vi "Get User Reference by Name.vi"(4 "error in (no error)":errorcluster, 6 "LoginName":string, 7 "EasyUserManager in":refnum<class "EasyUserManager.lvclass">) -> (0 "error out":errorcluster, 2 "User Reference":refnum<k7>, 3 "EasyUserManager out":refnum<class "EasyUserManager.lvclass">)   [LabVIEW 2024, in "EasyUserManager.lvclass"]
doc: "Returns the <B>User Reference</B> corresponding to the provided <B>LoginName</B>. \n\nYou must close the reference after using it."
uses:
  EasyUserManager.lvclass
  EasyUserManager.lvclass/EasyUserManager.ctl
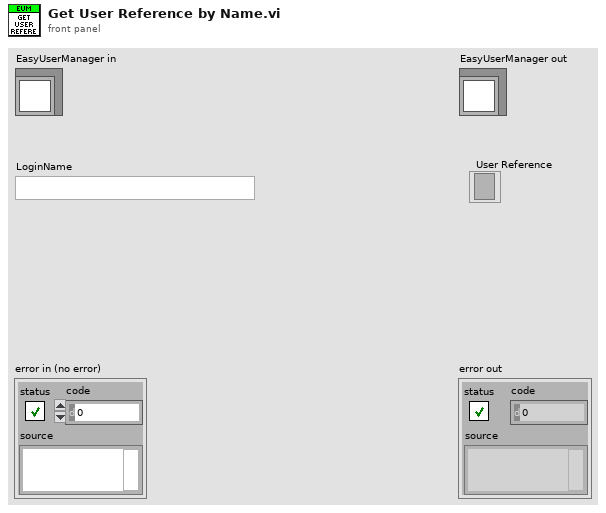
[diagram p1: front panel]
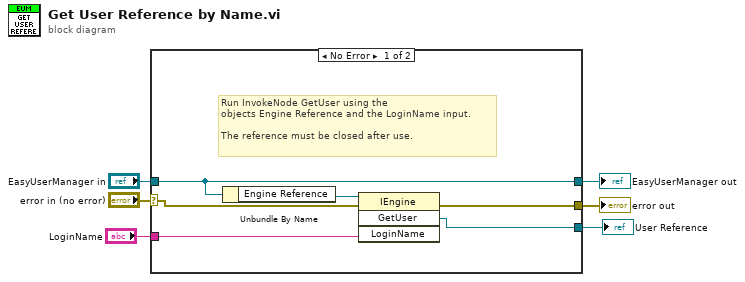
[diagram p0: block diagram]
diagram:
  n1 = case shown="No Error" "error in (no error)" {
    selector: "error in (no error)" -> [w9 w14]
    tunnel: [w10 w14] -> w5
    tunnel: [w12 w13] -> w3
    tunnel: "EasyUserManager in" -> [w12 w13]
    tunnel: "LoginName" -> [w8 _]
    tunnel: [w7 _] -> w1
    frame No Error {
      # "Run InvokeNode GetUser using the\nobjects Engine Reference and the LoginName input.\n\nThe reference must be closed after use."
      n2 = Unbundle By Name(w12) -> ("Engine Reference"=w11:refnum<k7>)
      n3 = invoke on="Invoke Node" class="IEngine" method="GetUser"(reference=w11, error in=w9, "LoginName"=w8) -> (error out=w10:errorcluster, "GetUser"=w7:refnum<k7>)  [unwired: 1 in, 2 out]
    }
    frame Error {
      # "Pass error and do nothing."
    }
  }
  "error out" <- w5
  "EasyUserManager out" <- w3
  "User Reference" <- w1
